vi "Progress Bar Example.vi"() -> ()   [LabVIEW 2015]
doc: "This example VI illustrates basic implementation of progress bar with 2 common patterns : fixed steps count and unknown steps count."
uses:
  <vilib>/Utility/sysdir.llb/System Directory Type.ctl
  Library/New Job Status.vi
  Library/New Item Status.vi
  Library/New Item Progression.vi
  Library/Class/Finish.vi
  Library/Class/Bar.lvclass
  Library/Simple Progress Bar.lvlib
panel:
  out "Process Error":errorcluster
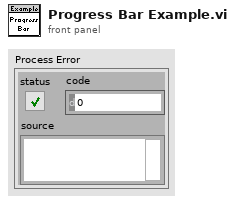
[diagram p1: front panel]
types:
  T1 = typedef "System Directory Type.ctl" = i32
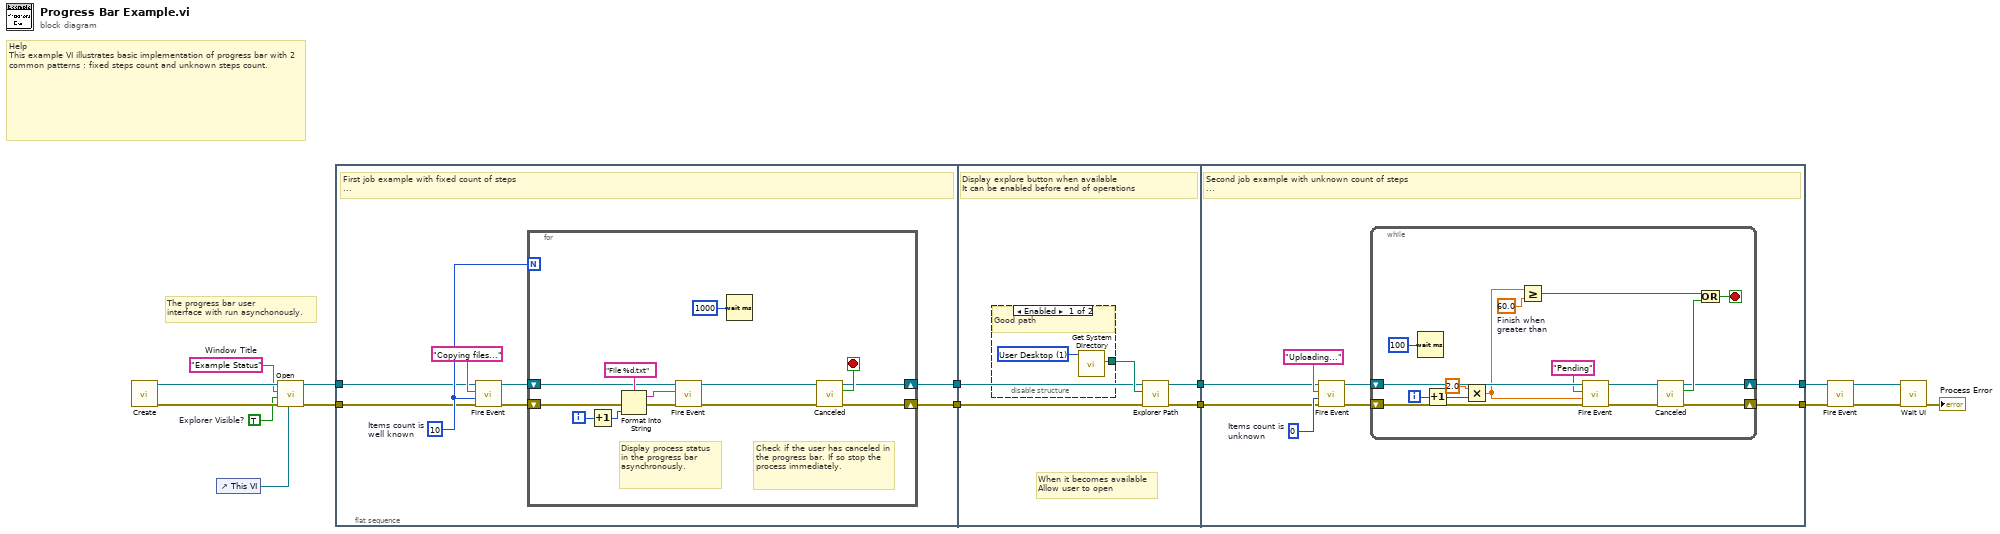
[diagram p0: block diagram]
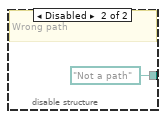
[diagram p2: hidden frame]
diagram:
  w9 = "Example Status"  # Window Title
  w11 = TRUE  # Explorer Visible?
  # "Help\nThis example VI illustrates basic implementation of progress bar with 2 common patterns : fixed steps count and unknown steps count."
  # "The progress bar user \ninterface with run asynchonously."
  n1 = call "Create.vi"() -> ("error out"=w14:errorcluster, "Bar out"=w10:refnum<class "Bar.lvclass">)  [unwired: 10 in]
  n2 = control-ref of="This VI"() -> (w12:refnum<vi>)
  n3 = call "Open.vi"("Caller VI"=w12, "error in (no error)"=w14, "Explorer Visible? (F)"=w11, "Window Title"=w9, "Bar in"=w10) -> ("error out"=w13:errorcluster, "Bar out"=w8:refnum<class "Bar.lvclass">)  [unwired: 5 in]
  n4 = flat-sequence {
    tunnel: w8 -> [w18]
    tunnel: w13 -> [w17]
    tunnel: [w20] -> w6
    tunnel: [w19] -> w5
    tunnel: w6 -> [w41]
    tunnel: w5 -> [w39]
    tunnel: [w40] -> w4
    tunnel: [w38] -> w3
    tunnel: [w46] -> w1
    tunnel: [w47] -> w2
    tunnel: w4 -> [w49]
    tunnel: w3 -> [w48]
    frame #0 {
      w22 = 10  # Items count is  well known
      # "First job example with fixed count of steps\n..."
      n5 = call-poly "Fire Event.vi"("error in (no error)"=w17, "Items Count (unknown)"=w22, "Status"="Copying files...", "Bar in"=w18) -> ("error out"=w23:errorcluster, "Bar out"=w24:refnum<class "Bar.lvclass">)  [unwired: 6 in]
      n6 = for {
        N: w22 -> [_]
        shift-right: [w28] -> w20
        shift-left: w23 -> [w37]
        shift-right: [w25] -> w19
        shift-left: w24 -> [w31]
        i -> [w36]
        stop <- w27 stop-if-true
        # "Check if the user has canceled in the progress bar. If so stop the process immediately."
        # "Display process status in the progress bar asynchronously."
        n7 = Increment(x=w36) -> (x+1=w35:i32)
        n8 = Format Into String(format string="File %d.txt", error in=w37, w35) -> (resulting string=w30:string, error out=w32:errorcluster)  [unwired: 1 in]
        n9 = call-poly "Fire Event.vi"("error in (no error)"=w32, "Status"=w30, "Bar in"=w31) -> ("error out"=w29:errorcluster, "Bar out"=w26:refnum<class "Bar.lvclass">)  [unwired: 7 in]
        n10 = Wait (ms)(milliseconds to wait=u32 1000) -> ()  [unwired: 1 out]
        n11 = call "Canceled.vi"("error in (no error)"=w29, "Bar in"=w26) -> ("error out"=w28:errorcluster, "Canceled by user?"=w27:bool, "Bar out"=w25:refnum<class "Bar.lvclass">)  [unwired: 7 in]
      }
    }
    frame #1 {
      # "When it becomes available\nAllow user to open"
      # "Display explore button when available\nIt can be enabled before end of operations"
      n12 = disable-structure shown="Enabled" {
        disable-tunnel: [w43 path "Not a path" ("Explorer Path")] -> w42
        frame Enabled {
          w44 = T1 1 items=["User Home"=0, "User Desktop"=1, "User Documents"=2, "User Application Data"=3, "User Preferences"=4, "User Temporary"=5, "Public Documents"=6, "Public Application Data"=7, "Public Preferences"=8, "Public Cache"=13, "System Core Libraries"=9, "System Installed Libraries"=10, "Application Files"=11, "Boot Volume Root"=12] ("system directory type")
          # "Good path"
          n13 = call <vilib>:"Get System Directory.vi"("system directory type"=w44) -> ("system directory"=w43:path)  [unwired: 10 in]
        }
        frame Disabled {
          # "Wrong path"
        }
      }
      n14 = call "Explorer Path.vi"("error in (no error)"=w41, "Explorer Path"=w42, "Bar in"=w39) -> ("error out"=w40:errorcluster, "Bar out"=w38:refnum<class "Bar.lvclass">)  [unwired: 7 in]
    }
    frame #2 {
      w50 = 0  # Items count is  unknown
      # "Second job example with unknown count of steps\n..."
      n15 = call-poly "Fire Event.vi"("error in (no error)"=w49, "Items Count (unknown)"=w50, "Status"="Uploading...", "Bar in"=w48) -> ("error out"=w52:errorcluster, "Bar out"=w53:refnum<class "Bar.lvclass">)  [unwired: 6 in]
      n16 = while {
        shift-right: [w59] -> w47
        shift-left: w52 -> [w65]
        shift-right: [w55] -> w46
        shift-left: w53 -> [w64]
        i -> [w67]
        stop <- w58 stop-if-true
        w61 = 60.0  # Finish when  greater than
        n17 = Wait (ms)(milliseconds to wait=u32 100) -> ()  [unwired: 1 out]
        n18 = Increment(x=w67) -> (x+1=w66:i32)
        n19 = Multiply(x=2.0, y=w66) -> (x*y=w62:dbl)
        n20 = Greater Or Equal?(x=w62, y=w61) -> (x >= y?=w60:bool)
        n21 = call-poly "Fire Event.vi"("error in (no error)"=w65, "Progression"=w62, "Status"="Pending", "Bar in"=w64) -> ("error out"=w54:errorcluster, "Bar out"=w56:refnum<class "Bar.lvclass">)  [unwired: 6 in]
        n22 = call "Canceled.vi"("error in (no error)"=w54, "Bar in"=w56) -> ("error out"=w59:errorcluster, "Canceled by user?"=w57:bool, "Bar out"=w55:refnum<class "Bar.lvclass">)  [unwired: 7 in]
        n23 = Or(x=w60, y=w57) -> (x .or. y?=w58:bool)
      }
    }
  }
  n24 = call-poly "Fire Event.vi"("error in (no error)"=w2, "Bar in"=w1) -> ("error out"=w15:errorcluster, "Bar out"=w7:refnum<class "Bar.lvclass">)  [unwired: 8 in]
  n25 = call "Wait UI.vi"("error in (no error)"=w15, "Bar in"=w7) -> ("error out"=→"Process Error":errorcluster)  [unwired: 6 in, 3 out]
